vi "IdentifyDropoff.vi"   [LabVIEW 2016, in "13.03 Robot.lvrbt"]
uses:
  13.03 Robot.lvrbt
  <vilib>/NXT/Dual Mode Library/Sensors/EV3_Color_Color.vi
  <vilib>/NXT/Subs/ColorSensorColors.ctl
  <vilib>/NXT/LegoClasses/BrickReference/BrickReference.lvclass
  <vilib>/NXT/Subs/LVHSConnector.ctl
  <vilib>/NXT/NXTIO Xnodes/NXTIOXNode/NXTIO.xnode
  <vilib>/NXT/NXTIO Xnodes/AddressXNode/NXTIOAddress.xnode
  <vilib>/NXT/Block Support/NXT_OutputPort.ctl
  <vilib>/NXT/NXTIO Xnodes/NXTIONodeSubVIs/NXTStopMotors.vi
  <vilib>/NXT/NXTIO Xnodes/NXTIONodeSubVIs/NXTMoveMotors.vi
types:
  T1 = typedef "NXT_OutputPort.ctl" = u8
  T2 = typedef "ColorSensorColors.ctl" = enum16{"No Color", "Black", "Blue", "Green", "Yellow", "Red", "White", "Brown"}
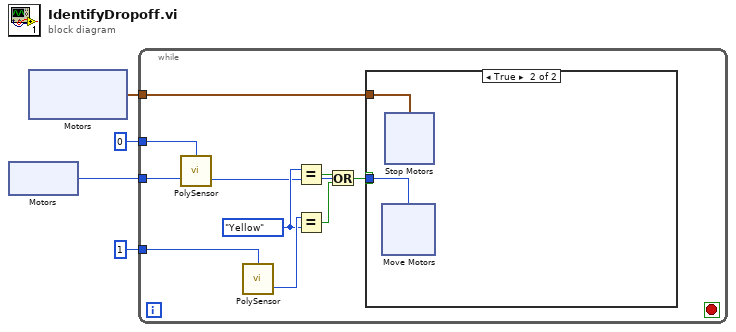
[diagram p0: block diagram]
diagram:
  n1 = xnode "Motors"() -> ("Motor"=w1:T1)
  n2 = xnode "Motors"() -> ("Motor"=w4:cluster{"Port":T1, "Port":T1})
  n3 = while {
    tunnel: 1 ("index") -> [w14]
    tunnel: w4 -> [w8]
    tunnel: 0 ("index") -> [w6]
    tunnel: w1 -> [w5]
    stop <- _ stop-if-true
    w11 = ColorSensorColors."Yellow" ("y")
    n4 = call-poly <vilib>:"PolySensor.vi"("Port (Port 1)"=w6) -> ("Detected Color"=w10:T2)  [unwired: 2 in, 1 out]
    n5 = call-poly <vilib>:"PolySensor.vi"("Port (Port 1)"=w14) -> ("Detected Color"=w13:T2)  [unwired: 2 in, 1 out]
    n6 = Equal?(x=w11, y=w10) -> (x = y?=w9:bool)
    n7 = Equal?(x=w13, y=w11) -> (x = y?=w12:bool)
    n8 = Or(x=w9, y=w12) -> (x .or. y?=w7:bool)
    n9 = case shown="True" w7 {
      tunnel: w8 -> [_ w16]
      tunnel: w5 -> [_ w15]
      frame False {
      }
      frame True {
        n10 = xnode "Move Motors"("Motors"=w15) -> ()  [unwired: 2 in, 1 out]
        n11 = xnode "Stop Motors"("Motors"=w16) -> ()  [unwired: 1 in, 1 out]
      }
    }
  }
